vi "Test Crop.vi"() -> ()   [LabVIEW 2017, in "Image Processing Library.lvlib"]
uses:
  Image Processing Library.lvlib
panel:
  in  "height":sgl=0.54
  in  "width":sgl=0.54
  in  "center_y":sgl=0.415
  in  "center_x":sgl=0.53
  out "Image Crop":picture
  out "Image In":picture
  out "error out":errorcluster
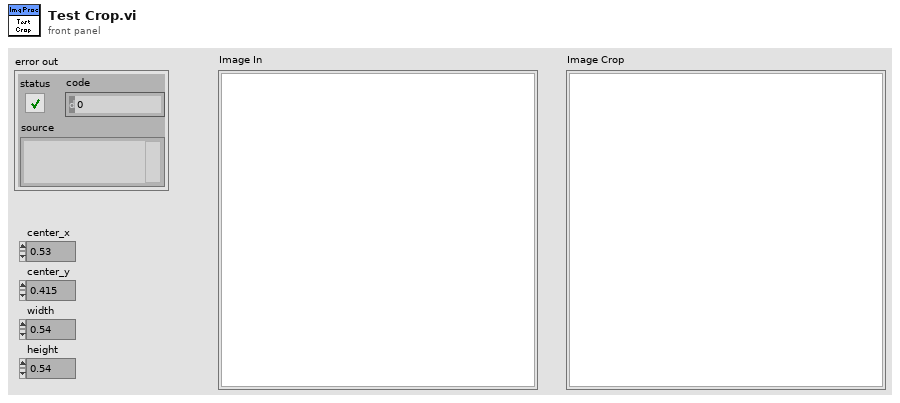
[diagram p1: front panel]
types:
  T1 = typedef "imagedata.ctl" = cluster{"image type":i32, "image depth":i32, "image":u8[], "mask":u8[], "colors":u32[], "Rectangle":cluster{"left":i16, "top":i16, "right":i16, "bottom":i16}}
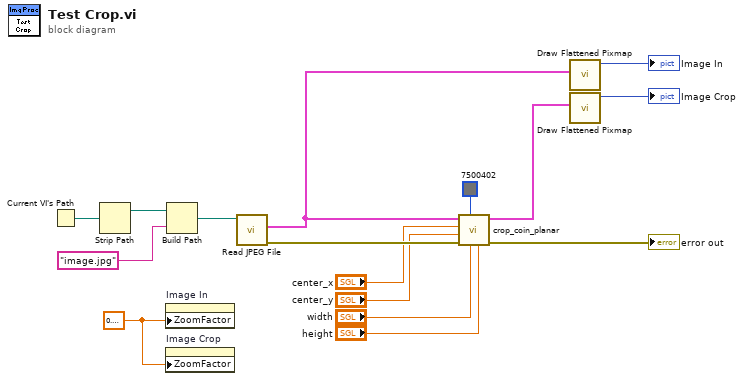
[diagram p0: block diagram]
diagram:
  w7 = sgl 0.3 ("Zoom Factor")
  n1 = Current VI's Path() -> (path=w15:path)
  n2 = Strip Path(path=w15) -> (stripped path=w14:path)  [unwired: 1 out]
  n3 = property on="Image In" class="Pict"("ZoomFactor"=w7) -> ()  [unwired: 2 in, 2 out]
  n4 = property on="Image Crop" class="Pict"("ZoomFactor"=w7) -> ()  [unwired: 2 in, 2 out]
  n5 = Build Path(base path=w14, name or relative path="image.jpg") -> (appended path=w13:path)
  n6 = call <vilib>:"Read JPEG File.vi"("path to JPEG file"=w13) -> ("error out"=w12:errorcluster, "image data"=w10:T1)  [unwired: 8 in, 1 out]
  n7 = call "crop_coin_planar.vi"("height"="height", "width"="width", "pad Color"=u32 7500402, "error in (no error)"=w12, "center_y"="center_y", "center_x"="center_x", "image in"=w10) -> ("error out"=→"error out":errorcluster, "image out"=w5:T1)  [unwired: 2 in, 1 out]
  n8 = call <vilib>:"Draw Flattened Pixmap.vi"("image data"=w10) -> ("new picture"=→"Image In":picture)  [unwired: 8 in]
  n9 = call <vilib>:"Draw Flattened Pixmap.vi"("image data"=w5) -> ("new picture"=→"Image Crop":picture)  [unwired: 8 in]
